vi "Missing VIs or controls on LV project.vi"(8 "error in (no error)":errorcluster, 11 "Path":path) -> (0 "error out":errorcluster, 3 "Pass":bool)   [LabVIEW 2021]
uses:
  <vilib>/addons/_JKI Toolkits/Caraya/classes/Assert/Assert False.vi
  <vilib>/addons/_JKI Toolkits/Caraya/classes/Test/Test.lvclass
  <vilib>/addons/_JKI Toolkits/Caraya/classes/Assert/Assert.lvclass
panel:
  out "Missing items from LabVIEW project":path[](array[path])
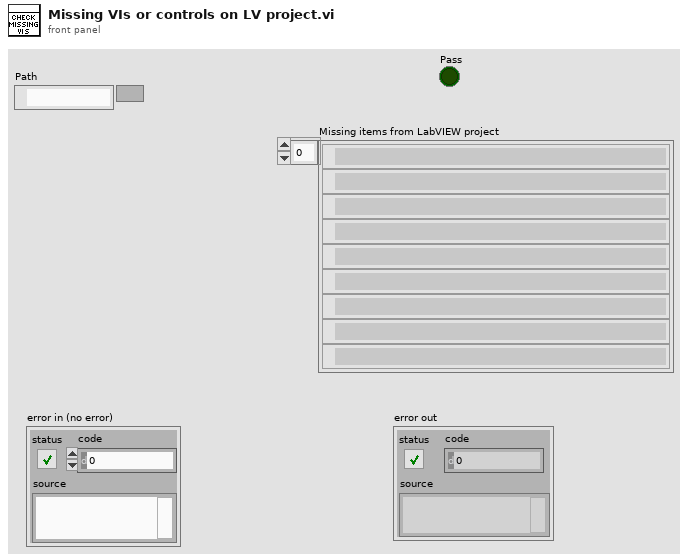
[diagram p1: front panel]
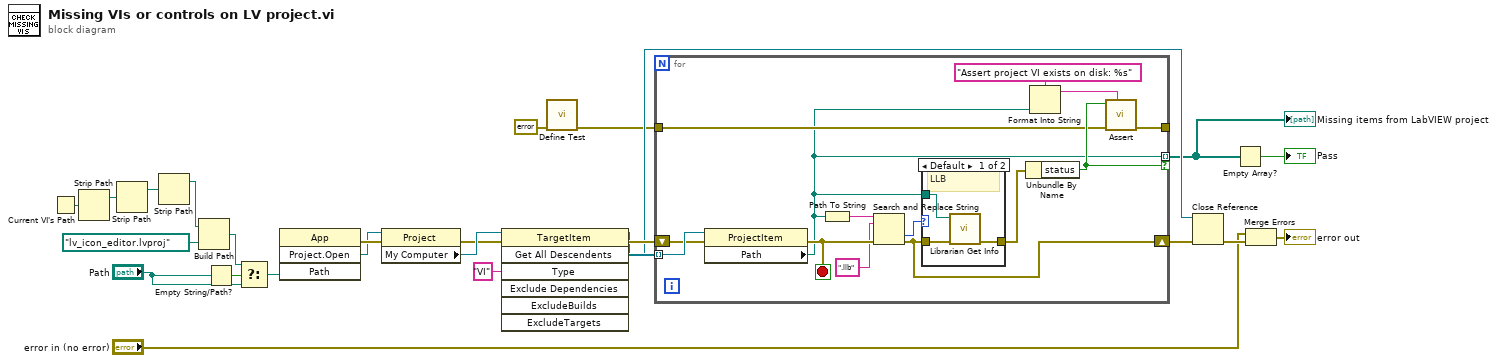
[diagram p0: block diagram]
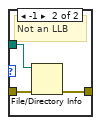
[diagram p2: hidden frame]
diagram:
  n1 = Current VI's Path() -> (path=w6:path)
  n2 = Strip Path(path=w6) -> (stripped path=w5:path)  [unwired: 1 out]
  n3 = Strip Path(path=w5) -> (stripped path=w4:path)  [unwired: 1 out]
  n4 = Strip Path(path=w4) -> (stripped path=w3:path)  [unwired: 1 out]
  n5 = Build Path(base path=w3, name or relative path=path "lv_icon_editor.lvproj") -> (appended path=w7:path)
  n6 = Empty String/Path?(string/path="Path") -> (empty?=w8:bool)
  n7 = Select(t=w7, s=w8, f="Path") -> (s? t:f=w2:path)
  n8 = invoke on="Invoke Node" class="App" method="Project.Open"("Path"=w2) -> (error out=w18:errorcluster, "Project:Open"=w17:refnum<vi>)  [unwired: 3 in, 2 out]
  n9 = property on="Property Node" class="Project"(reference=w17, error in=w18) -> (error out=w22:errorcluster, "My Computer"=w25:refnum<vi>)  [unwired: 1 out]
  n10 = invoke on="Invoke Node" class="TargetItem" method="Get All Descendents"(reference=w25, error in=w22, "Type"="VI") -> (reference out=w19:refnum<vi>, error out=w21:errorcluster, "All Descendents"=w23:refnum<vi>[])  [unwired: 4 in, 4 out]
  n11 = call <vilib>:"Define Test.vi"("error in (no error)"=errorcluster {"status"=FALSE, "code"=0, "source"=""}) -> ("error out"=w10:errorcluster)  [unwired: 9 in, 1 out]
  n12 = for {
    tunnel: w23 -> [w39] mode=indexing
    shift-right: [w26] -> w20
    shift-left: w21 -> [w38]
    tunnel: [w27] -> w16 mode=indexing if=w37
    tunnel: w10 -> [w36]
    tunnel: [w33] -> _
    stop <- w32 stop-if-true
    n13 = property on="Property Node" class="ProjectItem"(reference=w39, error in=w38) -> (error out=w32:errorcluster, "Path"=w27:path)  [unwired: 1 out]
    n14 = Path To String(path=w27) -> (string=w31:string)
    n15 = Search and Replace String(input string=w31, search string=".llb", error in=w32) -> (offset past replacement=w29:i32, error out=w26:errorcluster)  [unwired: 5 in, 2 out]
    n16 = case shown="Default" w29 {
      tunnel: w26 -> [w42 w45]
      tunnel: [w41 w44] -> w28
      tunnel: w27 -> [w40 w43]
      frame Default {
        # "LLB"
        n17 = call <vilib>:"Librarian Get Info.vi"("error in (no error)"=w42, "path"=w40) -> ("error out"=w41:errorcluster)  [unwired: 7 in, 2 out]
      }
      frame -1 {
        # "Not an LLB"
        n18 = File/Directory Info(path=w43, error in=w45) -> (error out=w44:errorcluster)  [unwired: 6 out]
      }
    }
    n19 = Unbundle By Name(w28) -> ("status"=w37:bool)
    n20 = Format Into String(format string="Assert project VI exists on disk: %s" ("Label"), w27) -> (resulting string=w34:string)  [unwired: 2 in, 1 out]
    n21 = call-poly <vilib>:"Assert.vi"("Label"=w34, "error in (no error)"=w36, "False?"=w37) -> ("error out"=w33:errorcluster)  [unwired: 7 in, 1 out]
  }
  "Missing items from LabVIEW project" <- w16
  n22 = Close Reference(reference=w19, error in (no error)=w20) -> (error out=w15:errorcluster)
  n23 = Empty Array?(array=w16) -> (empty?=→"Pass":bool)
  n24 = Merge Errors("error in (no error)", w15) -> (→"error out":errorcluster)
